vi "Verification_programme EPC3000.vi"(1 "Programme_entrée":cluster{"chaîne":string, "Valeur":dbl}[][](array[cluster]) {"Valeur" format="%#.1f"}) -> (0 "Programme_sortie":cluster{"chaîne":string, "Valeur":dbl}[][](array[cluster]) {"Valeur" format="%#.1f"})   [LabVIEW 2022 SP3]
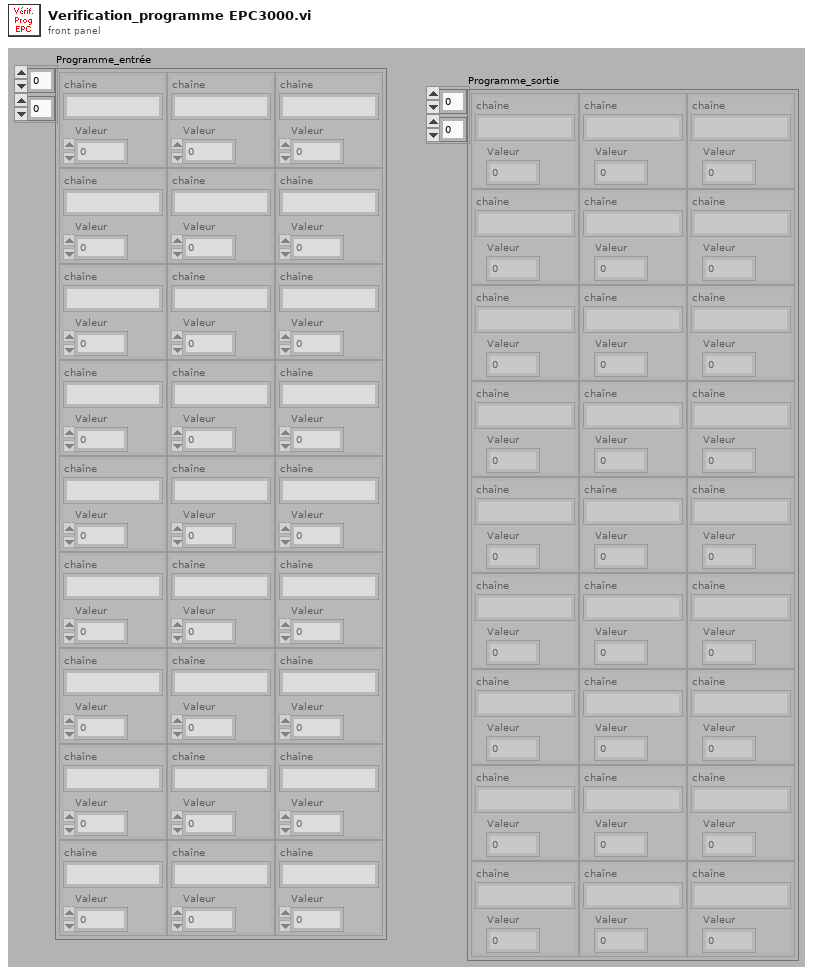
[diagram p1: front panel]
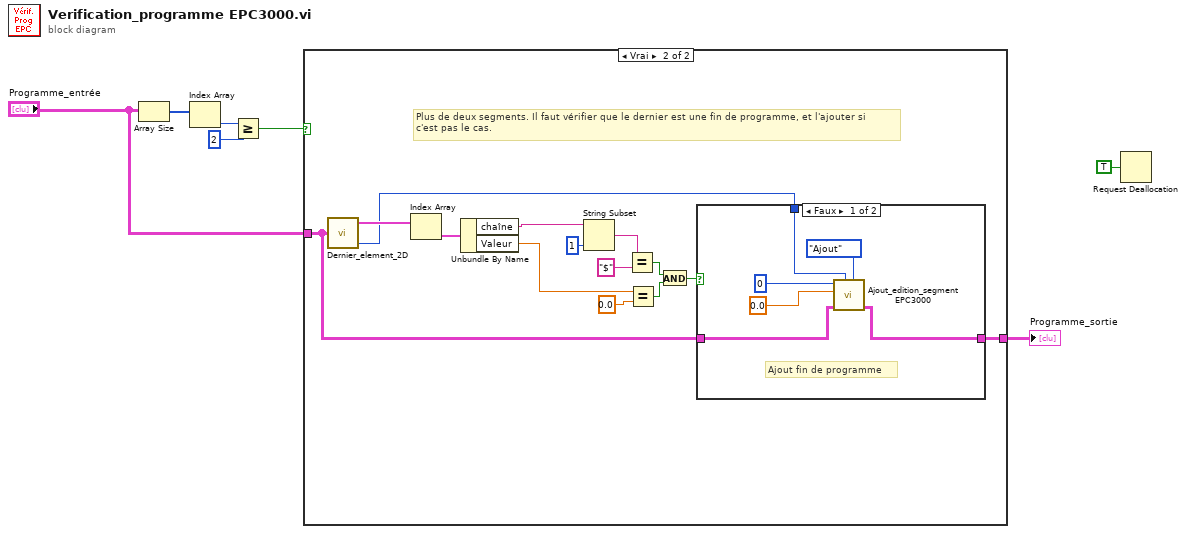
[diagram p0: block diagram]
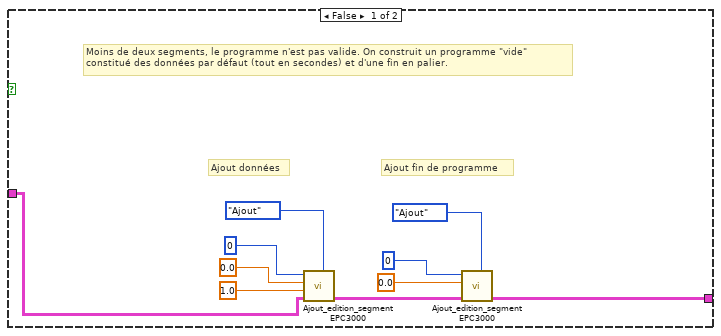
[diagram p2: hidden frame]
diagram:
  n1 = Array Size(array="Programme_entrée") -> (size(s)=w7:i32[])
  n2 = Index Array(array=w7) -> (element=w6:i32)  [unwired: 1 in]
  n3 = Greater Or Equal?(x=w6, y=2) -> (x >= y?=w4:bool)
  n4 = case shown="Vrai" w4 {
    tunnel: "Programme_entrée" -> [w10 w20]
    tunnel: [w11 w19] -> w3
    frame False {
      # "Ajout données"
      # "Ajout fin de programme"
      # "Moins de deux segments, le programme n'est pas valide. On construit un programme \"vide\"\nconstitué des données par défaut (tout en secondes) et d'une fin en palier."
      n5 = call "Ajout_edition_segment EPC3000.vi"("Action"=enum16{"Edition", "Insertion", "Ajout"}."Ajout", "Programme_entrée"=w10, "Valeur 2"=1.0, "Valeur 1"=0.0, "Type de segment/Valeur 0"=u8 0) -> ("Programme_sortie"=w12:cluster{"chaîne":string, "Valeur":dbl}[][])  [unwired: 6 in]
      n6 = call "Ajout_edition_segment EPC3000.vi"("Action"=enum16{"Edition", "Insertion", "Ajout"}."Ajout", "Programme_entrée"=w12, "Valeur 1"=0.0, "Type de segment/Valeur 0"=u8 0) -> ("Programme_sortie"=w11:cluster{"chaîne":string, "Valeur":dbl}[][])  [unwired: 7 in]
    }
    frame True {
      # "Plus de deux segments. Il faut vérifier que le dernier est une fin de programme, et l'ajouter si\nc'est pas le cas."
      n7 = call "Dernier_element_2D.vi"("Programme"=w20) -> ("Dernier segment"=w31:cluster{"chaîne":string, "Valeur":dbl}[], "Taille/Indice N+1"=w18:i32)  [unwired: 1 out]
      n8 = Index Array(array=w31) -> (element=w30:cluster{"chaîne":string, "Valeur":dbl})  [unwired: 1 in]
      n9 = Unbundle By Name(w30) -> ("chaîne"=w25:string, "Valeur"=w24:dbl)
      n10 = String Subset(string=w25, length (rest)=1 ("longueur (reste)")) -> (substring=w27:string)  [unwired: 1 in]
      n11 = Equal?(x=w27, y="$") -> (x = y?=w23:bool)
      n12 = Equal?(x=w24, y=0.0) -> (x = y?=w22:bool)
      n13 = And(x=w23, y=w22) -> (x .and. y?=w21:bool)
      n14 = case shown="Faux" w21 {
        tunnel: w20 -> [w37 w38]
        tunnel: [w36 w38] -> w19
        tunnel: w18 -> [w35 _]
        frame False {
          # "Ajout fin de programme"
          n15 = call "Ajout_edition_segment EPC3000.vi"("Action"=enum16{"Edition", "Insertion", "Ajout"}."Ajout", "Numéro du segment"=w35, "Programme_entrée"=w37, "Valeur 1"=0.0, "Type de segment/Valeur 0"=u8 0) -> ("Programme_sortie"=w36:cluster{"chaîne":string, "Valeur":dbl}[][])  [unwired: 6 in]
        }
        frame True {
          # "Fin de programme présente - OK !"
        }
      }
    }
  }
  "Programme_sortie" <- w3
  n16 = Request Deallocation(TRUE ("flag")) -> ()
